vi "DAC Run.vi"(8 "error in":errorcluster, 11 "DAC Pump Inv in":refnum<class "DAC Pump Inv.lvclass">) -> (0 "error out":errorcluster, 3 "DAC Pump Inv out":refnum<class "DAC Pump Inv.lvclass">)   [LabVIEW 2019, in "DAC.lvlib" / "DAC Pump Inv.lvclass"]
uses:
  DAC Pump Inv.lvclass
  C:/Users/wg/Documents/LV_Projects/test-stand/App/DAC/DAC.lvclass
  DAC.lvclass/DAC.ctl
  Results/Results Method.ctl
  Results/Water Tunnel Results/Water Tunnel Results.lvclass
  DAC Pump Inv.lvclass/DAC Pump Inv.ctl
  <vilib>/DAQmx/write.llb/DAQmx Write (Analog DBL 1Chan 1Samp).vi
  <vilib>/DAQmx/miscellaneous.llb/DAQmx Fill In Error Info.vi
  DAC.lvclass
  Results/Results.lvlib
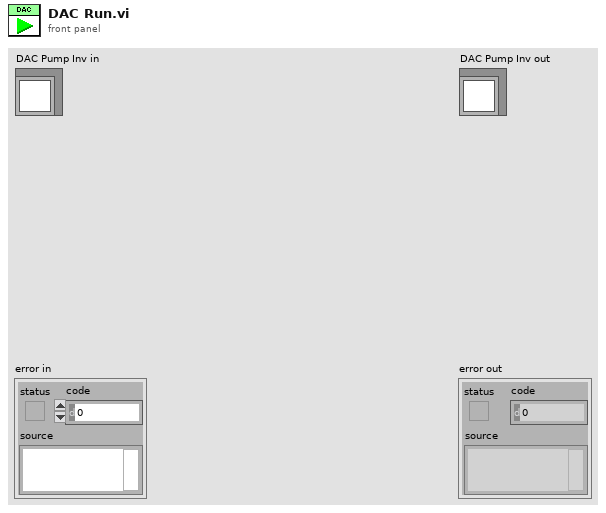
[diagram p1: front panel]
types:
  T1 = typedef "Results.lvlib/Results Method.ctl" = enum16{"Get", "Set"}
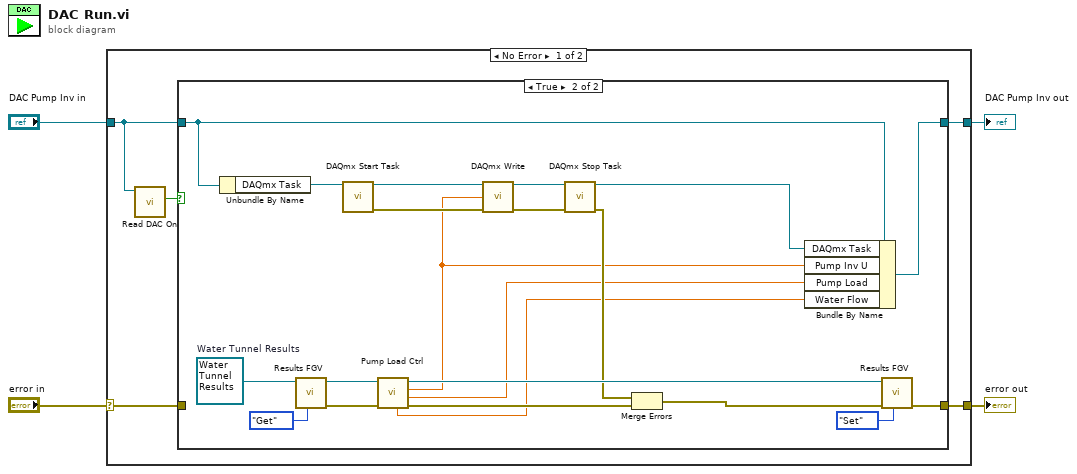
[diagram p0: block diagram]
diagram:
  n1 = case shown="No Error" "error in" {
    selector: "error in" -> [w7 w34]
    tunnel: [w6 w34] -> w2
    tunnel: [w8 w33] -> w1
    tunnel: "DAC Pump Inv in" -> [w5 w33]
    frame No Error {
      n2 = call "Read DAC On.vi"("DAC in"=w5) -> ("DAC On"=w9:bool)  [unwired: 8 in, 2 out]
      n3 = case shown="True" w9 {
        tunnel: w5 -> [w11 w28]
        tunnel: [w11 w23] -> w8
        tunnel: w7 -> [w10 _]
        tunnel: [w10 w22] -> w6
        frame False {
        }
        frame True {
          w21 = refnum<class "Water Tunnel Results.lvclass"> refnum  # Water Tunnel Results
          n4 = Unbundle By Name(w28) -> ("DAQmx Task"=w32:refnum<k21>)
          n5 = call-dynamic "Results FGV.vi"("Method"=Results_Method."Get", "Water Tunnel Results in"=w21) -> ("error out"=w18:errorcluster, "Water Tunnel  Results out"=w20:refnum<class "Water Tunnel Results.lvclass">)  [unwired: 8 in]
          n6 = call <vilib>:"DAQmx Start Task.vi"("task/channels in"=w32) -> ("task out"=w31:refnum<k21>, "error out"=w30:errorcluster)  [unwired: 13 in]
          n7 = call "Pump Load Ctrl.vi"("error in"=w18, "Water Tunnel Results in"=w20) -> ("error out"=w16:errorcluster, "Pump Load"=w13:dbl, "Pump Inv U"=w14:dbl, "Water Tunnel Results out"=w19:refnum<class "Water Tunnel Results.lvclass">, "Water Flow"=w12:dbl)  [unwired: 5 in]
          n8 = call-poly <vilib>:"DAQmx Write.vi"("task/channels in"=w31, "data"=w14, "error in"=w30) -> ("task out"=w24:refnum<k21>, "error out"=w29:errorcluster)  [unwired: 10 in, 1 out]
          n9 = call <vilib>:"DAQmx Stop Task.vi"("task/channels in"=w24, "error in"=w29) -> ("task out"=w25:refnum<k21>, "error out"=w17:errorcluster)  [unwired: 12 in]
          n10 = Merge Errors(w17, w16) -> (w15:errorcluster)
          n11 = Bundle By Name(cluster=w28, "DAQmx Task"=w25, "Pump Inv U"=w14, "Pump Load"=w13, "Water Flow"=w12) -> (w23:refnum<class "DAC Pump Inv.lvclass">)
          n12 = call-dynamic "Results FGV.vi"("Method"=Results_Method."Set", "error in"=w15, "Water Tunnel Results in"=w19) -> ("error out"=w22:errorcluster)  [unwired: 7 in, 1 out]
        }
      }
    }
    frame Error {
    }
  }
  "error out" <- w2
  "DAC Pump Inv out" <- w1
